vi "PIDAutoTune_ClosedLoopStep.vi"(7 "Configuration Parameters":T2={"Controller Constant Type"=enum."Ziegler Nicols - Normal", "Type of Controller"=enum."PI", "CO Offset"=0.25, "Kn"=1.0, "Tuning Tolerance"=0.001, "Plant Tolerance"=0.001, "Newest Avg Time "=1, "Long Ave Time"=6}, 8 "Sampling Time dt (s)":dbl=0.02, 9 "Tune":bool, 10 "Measurement  (PV)":dbl, 11 "Control Output (Co)":dbl) -> (0 "Plant and Test Data":T4, 1 "New Tuning Parameters":T3, 2 "Tuning Done":bool, 3 "Adj CO":dbl, 4 "Error Occured":bool, 6 "Diagnostic":T1)   [LabVIEW 2019, in "Trajectory_Library.lvlib"]
doc: "This routine can be used to make a step change to a PID control loop, track the results, and calculate PID tuning parameters. It wraps the NI LabVIEW PID auto-tuning functions for use with the WPILIB LabVIEW Math PID. This uses the CLOSED LOOP STEP type of test. \n\nWarning -- This routine will modify the control output. Use it in such a manner to be able to stop the tuning if problems occur -- like running out of field space while tuning a drive motor. \n\nInputs:\n -- Configuration Parameters -- cluster -- This contains the parameters defining the conditions of the test. Use the Pack routine to create this data cluster.\n -- Control Output -- double -- The Control Output (CO) value from the output of the PID to be tuned.\n -- Measurement (PV) -- double -- The Process Variable (PV) value used by the PID to be tuned.\n -- Tune -- boolean -- When TRUE, tuning is performed..\n -- Sampling time -- double -- Loop time in seconds. How fast the PID and this autotune function are executed. (Optional: Default 0.02 seconds) \n\nOutputs:\n -- Adj CO -- double -- The adjusted CO. This is sent to the actuator. (This vi is put between the PID and the actuator device)\n -- Tuning Done -- boolean -- This is set to TRUE when tuning has completed. Depending on the PV noise, tuning may never be \"DONE\". However if the new tuning parameters are relatively constant, they can still be used.\n -- New Tuning Parameters -- cluster --- Data cluster containing the calculated PID tuning parameters. \n -- Plant and Test Data -- cluster -- Data cluster containing information describing the transfer function of the system being controlled (Plant).\n -- Error Occured -- Boolean -- If TRUE, an error occured.\n -- Diagnostic Info -- cluster -- This contains additional information about the test being perfromed."
uses:
  Trajectory_Library.lvlib
  Timer_New.vi
  LinearFilter_ResetToValue.vi
  LinearFilter_Calculate.vi
  <vilib>/Utility/semaphor.llb/Obtain Semaphore Reference.vi
  Timer_Reset.vi
  Timer_Start.vi
  Timer_Stop.vi
  Timer_HasPeriodPassedOnce.vi
  <vilib>/addons/control/pid/autopid.llb/PID Autotuning Design (Auto).vi
  <vilib>/addons/control/pid/autopid.llb/PID Autotuning Design (Chien-Hrones-Reswick).vi
  LinearFilter_MovingAverage.vi
  LinearFilter_LowPassBW1.vi
  LinearFilter_LowPassBW2.vi
  LinearFilter_HighPassBW1.vi
  LinearFilter_HighPassBW2.vi
  <vilib>/Analysis/Matrix/Numeric/Conversions/Array To Matrix - RA.vi
  <vilib>/addons/control/pid/NI_PID_autopid.lvlib
  <vilib>/ptbypt/NI_PtbyPt.lvlib
  <vilib>/Analysis/Matrix/NI_Matrix.lvlib
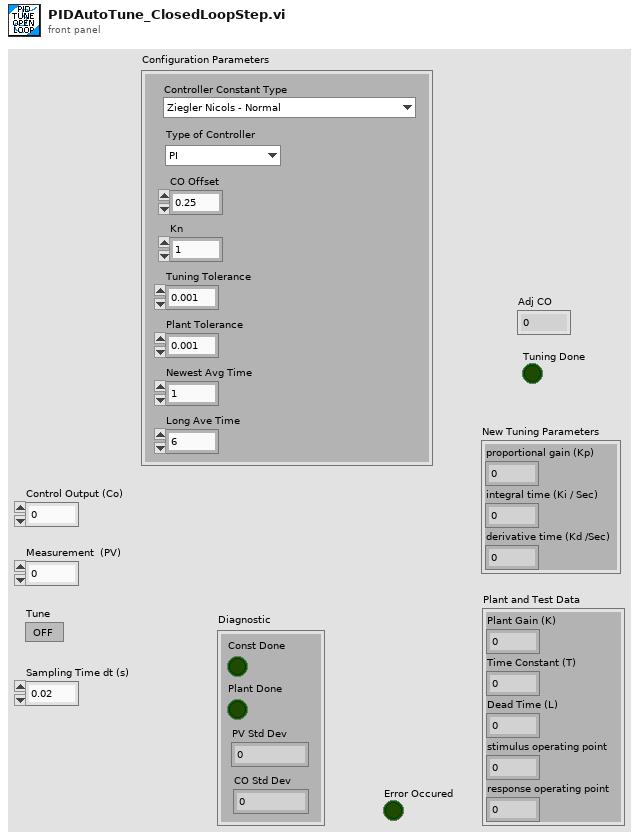
[diagram p1: front panel]
types:
  T1 = cluster{"Const Done":bool, "Plant Done":bool, "PV Std Dev":dbl, "CO Std Dev":dbl}
  T2 = cluster{"Controller Constant Type":enum16{"Ziegler Nicols - Fast", "Ziegler Nicols - Normal", "Ziegler Nicols - Slow", "CHR regulator - 0% overshoot", "CHR regulator - 20% overshoot", "CHR servo - 0 % overshoot", "CHR servo - 20% overshoot"}, "Type of Controller":enum16{"P", "PI", "PID"}, "CO Offset":dbl, "Kn":dbl, "Tuning Tolerance":dbl, "Plant Tolerance":dbl, "Newest Avg Time ":i32, "Long Ave Time":i32}
  T3 = cluster{"proportional gain (Kp)":dbl, "integral time (Ki / Sec)":dbl, "derivative time (Kd /Sec)":dbl}
  T4 = cluster{"Plant Gain (K)":dbl, "Time Constant (T)":dbl, "Dead Time (L)":dbl, "stimulus operating point":dbl, "response operating point":dbl}
  T5 = enum16{"Ziegler Nicols - Fast", "Ziegler Nicols - Normal", "Ziegler Nicols - Slow", "CHR regulator - 0% overshoot", "CHR regulator - 20% overshoot", "CHR servo - 0 % overshoot", "CHR servo - 20% overshoot"}
  T6 = cluster{"proportional gain (Kc)":dbl, "integral time (Ti, min)":dbl, "derivative time (Td, min)":dbl}
  T7 = cluster{"Plant Gain (K)":dbl, "Time Constant (T)":dbl, "Dead Time (L)":dbl}
  T8 = cluster{"Plant Gain (K)":dbl, "Time Constant (T)":dbl, "Dead Time (L)":dbl, "stimulus offset":dbl, "response offset":dbl}
  T9 = typedef "NI_Matrix.lvlib/RealMatrix.ctl" = dbl[][]
  T10 = cluster{"WithinTolerance":bool, "WithinTolerance":bool, "standard deviation":dbl, "standard deviation":dbl}
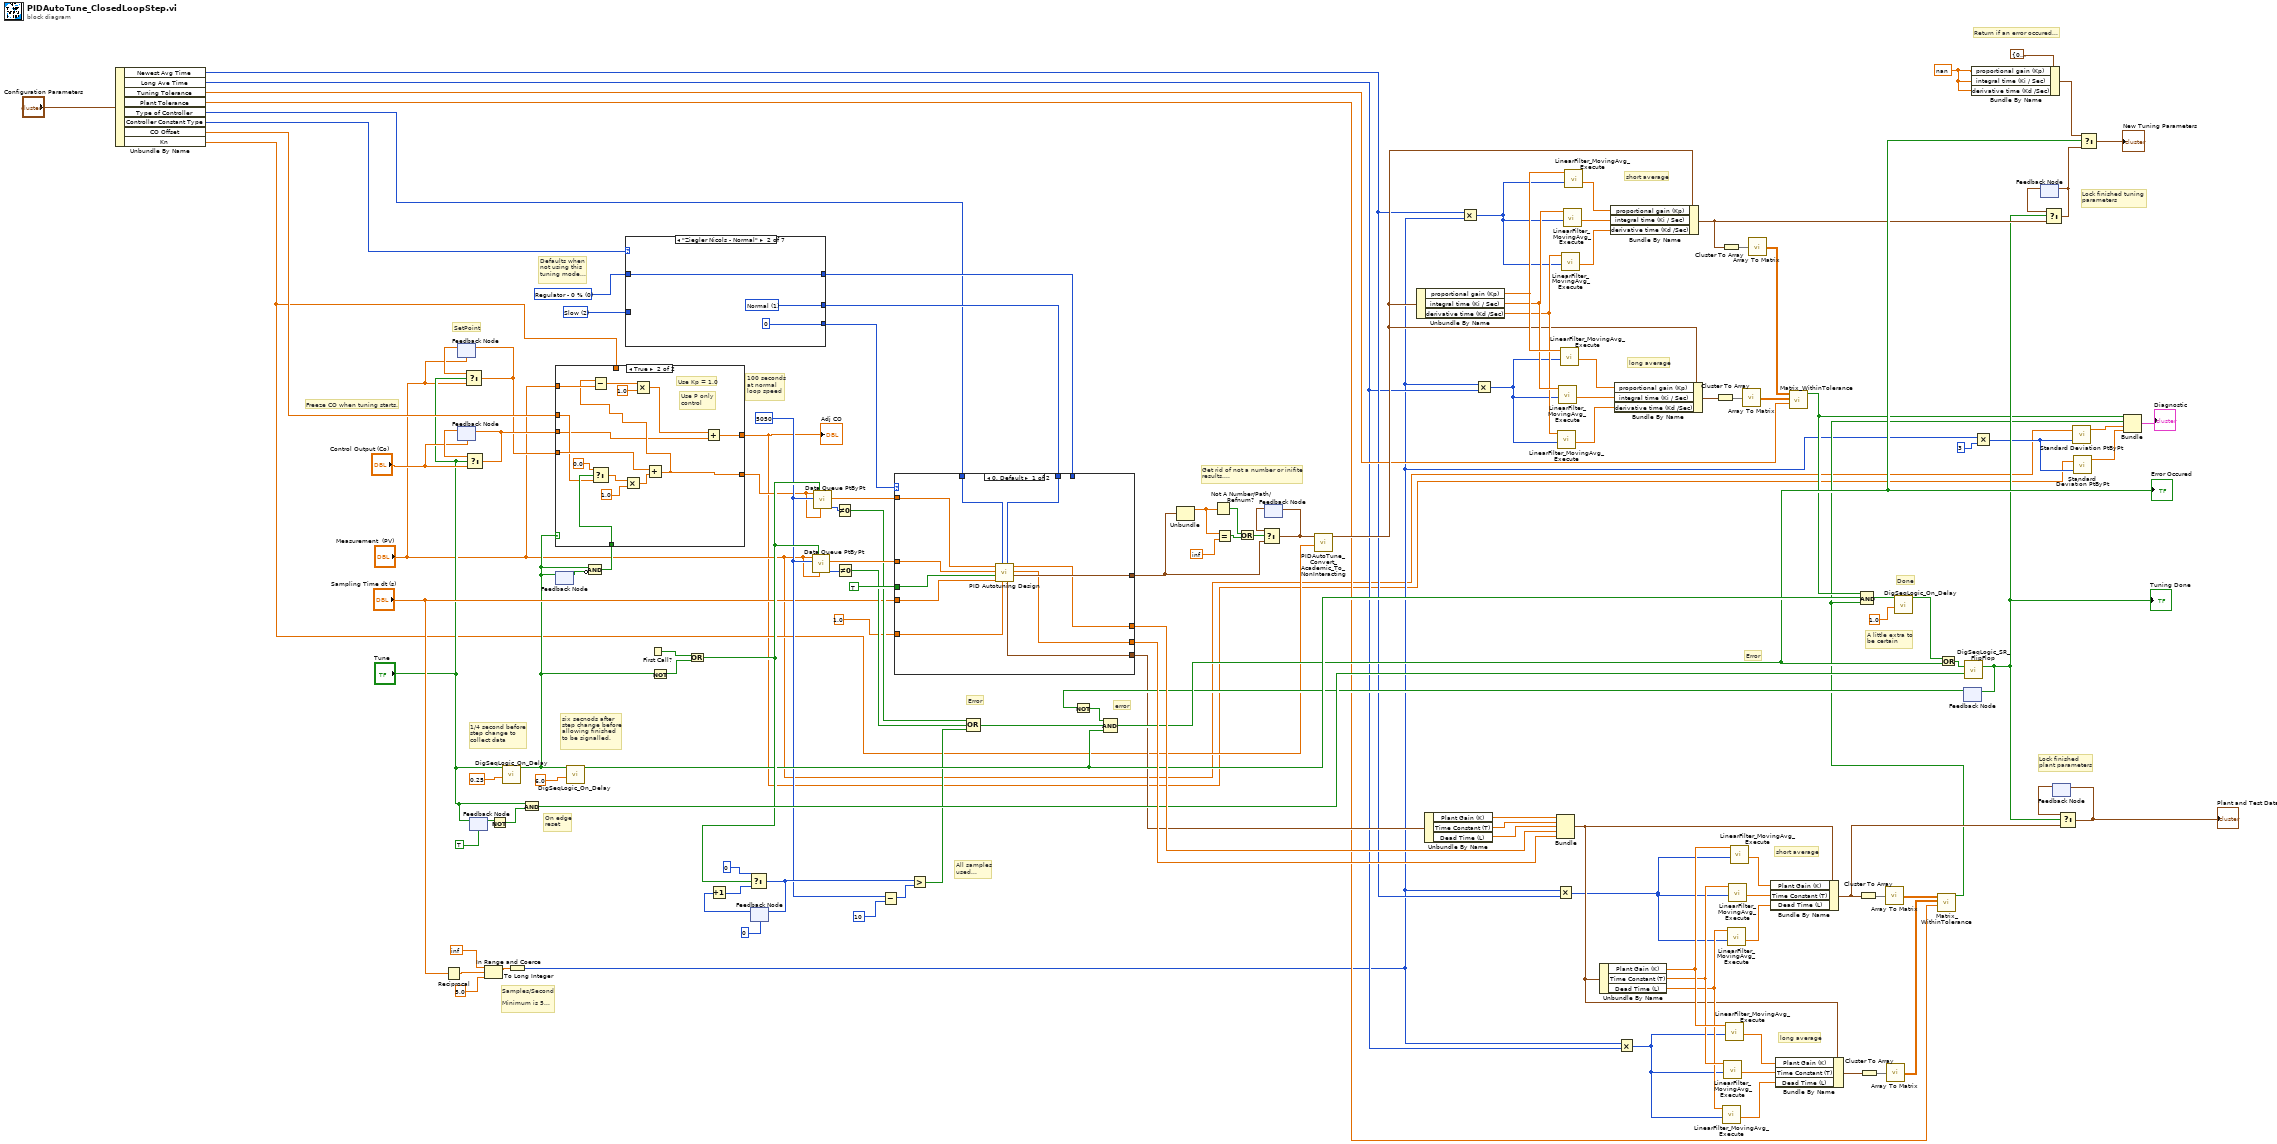
[diagram p0: block diagram]
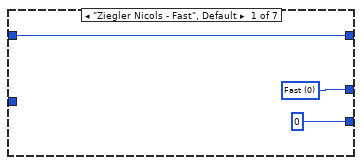
[diagram p2: hidden frame]
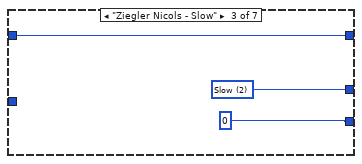
[diagram p3: hidden frame]
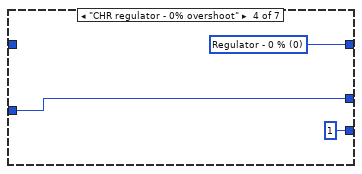
[diagram p4: hidden frame]
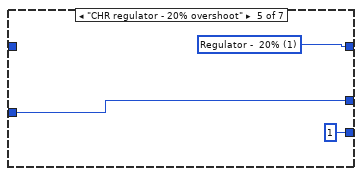
[diagram p5: hidden frame]
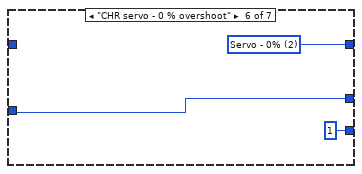
[diagram p6: hidden frame]
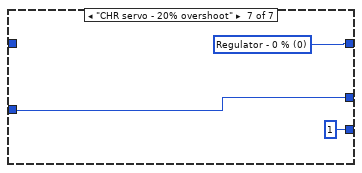
[diagram p7: hidden frame]
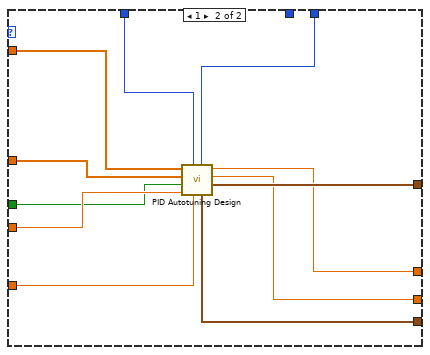
[diagram p8: hidden frame]
diagram:
  w89 = nan
  w104 = u16 2 items=["Fast", "Normal", "Slow"] ("Ziegler-Nichols Speed")
  w105 = u16 0 items=["Regulator - 0 %", "Regulator -  20%", "Servo - 0%", "Servo - 20%"] ("Tuning specifications")
  w76 = 5050 ("sample length")
  # "SetPoint"
  # "Get rid of not a number or inifite\nresults...."
  # "On edge\nreset"
  # "Error"
  # "All samples\nused..."
  # "Error"
  # "Done"
  # "Lock finished \nplant parameters"
  # "Lock finished tuning\nparameters"
  # "Samples/Second\n\nMinimum is 5..."
  # "long average"
  # "short average"
  # "long average"
  # "short average"
  # "error"
  # "Return if an error occured..."
  # "A little extra to\nbe certain"
  # "Defaults when\nnot using this\ntuning mode..."
  # "100 seconds\nat normal\nloop speed"
  # "Freeze CO when tuning starts."
  # "six secnods after\nstep change before\nallowing finished \nto be signalled."
  # "1/4 second before\nstep change to\ncollect data"
  n1 = Unbundle By Name("Configuration Parameters") -> ("Newest Avg Time"=w21:i32, "Long Ave Time"=w20:i32, "Tuning Tolerance"=w26:dbl, "Plant Tolerance"=w25:dbl, "Type of Controller"=w28:enum16{"P", "PI", "PID"}, "Controller Constant Type"=w29:T5, "CO Offset"=w27:dbl, "Kn"=w9:dbl)
  n2 = Reciprocal(x="Sampling Time dt (s)") -> (1/x=w66:dbl)
  n3 = feedback #1("Measurement  (PV)") -> (w16:dbl)
  n4 = feedback #2("Control Output (Co)") -> (w119:dbl)
  n5 = Select(t=w16, s="Tune", f="Measurement  (PV)") -> (s? t:f=w14:dbl)
  n6 = feedback-in #1(w14) -> ()
  n7 = Select(t=w119, s="Tune", f="Control Output (Co)") -> (s? t:f=w120:dbl)
  n8 = feedback-in #2(w120) -> ()
  n9 = feedback-in #3("Tune") -> ()
  n10 = feedback #3(TRUE ("Tune")) -> (w116:bool)
  n11 = In Range and Coerce(upper limit=inf, x=w66, lower limit=5.0) -> (coerced(x)=w57:dbl)  [unwired: 1 out]
  n12 = Not(x=w116) -> (.not. x?=w115:bool)
  n13 = call "DigSeqLogic_On_Delay.vi"("Delay"=0.25, "Input"="Tune") -> ("Output"=w10:bool)  [unwired: 8 in, 1 out]
  n14 = To Long Integer(number=w57) -> (32bit integer=w5:i32)
  n15 = And(x="Tune", y=w115) -> (x .and. y?=w114:bool)
  n16 = feedback-in #4(w10) -> ()
  n17 = feedback #4() -> (w13:bool)  [unwired: 1 in]
  n18 = call "DigSeqLogic_On_Delay.vi"("Delay"=6.0, "Input"=w10) -> ("Output"=w83:bool)  [unwired: 8 in, 1 out]
  n19 = Compound Arithmetic op=AND(w10, invert w13) -> (w12:bool)
  n20 = case shown="True" w10 {
    tunnel: w120 -> [w135 w140]
    tunnel: w27 -> [_ w141]
    tunnel: [w135 w146] -> w1
    tunnel: w14 -> [w134 w143]
    tunnel: "Measurement  (PV)" -> [_ w149]
    tunnel: w12 -> [_ w144]
    tunnel: [w134 w142] -> w11
    tunnel: w9 -> [_ _]
    frame False {
    }
    frame True {
      # "Use P only \ncontrol"
      # "Use Kp = 1.0"
      n21 = Select(t=0.0, s=w144, f=w141) -> (s? t:f=w137:dbl)
      n22 = Multiply(x=w137, y=1.0) -> (x*y=w139:dbl)
      n23 = Add(x=w143, y=w139) -> (x+y=w142:dbl)
      n24 = Subtract(x=w142, y=w149) -> (x-y=w148:dbl)
      n25 = Multiply(x=w148, y=1.0) -> (x*y=w147:dbl)
      n26 = Add(x=w147, y=w140) -> (x+y=w146:dbl)
    }
  }
  "Adj CO" <- w1
  n27 = case shown="\"Ziegler Nicols - Normal\"" w29 {
    tunnel: [w152 w155 w158 w159 w162 w165 w168] -> w108
    tunnel: [0 0 0 1 1 1 1] -> w107
    tunnel: [w150 w153 w156 w160 w163 w166 w169] -> w106
    tunnel: w105 -> [w150 w153 w156 _ _ _ _]
    tunnel: w104 -> [_ _ _ w159 w162 w165 w168]
    frame "Ziegler Nicols - Fast", Default {
      w152 = u16 0 items=["Fast", "Normal", "Slow"] ("Ziegler-Nichols Speed")
    }
    frame "Ziegler Nicols - Normal" {
      w155 = u16 1 items=["Fast", "Normal", "Slow"] ("Ziegler-Nichols Speed")
    }
    frame "Ziegler Nicols - Slow" {
      w158 = u16 2 items=["Fast", "Normal", "Slow"] ("Ziegler-Nichols Speed")
    }
    frame "CHR regulator - 0% overshoot" {
      w160 = u16 0 items=["Regulator - 0 %", "Regulator -  20%", "Servo - 0%", "Servo - 20%"] ("Tuning specifications")
    }
    frame "CHR regulator - 20% overshoot" {
      w163 = u16 1 items=["Regulator - 0 %", "Regulator -  20%", "Servo - 0%", "Servo - 20%"] ("Tuning specifications")
    }
    frame "CHR servo - 0 % overshoot" {
      w166 = u16 2 items=["Regulator - 0 %", "Regulator -  20%", "Servo - 0%", "Servo - 20%"] ("Tuning specifications")
    }
    frame "CHR servo - 20% overshoot" {
      w169 = u16 0 items=["Regulator - 0 %", "Regulator -  20%", "Servo - 0%", "Servo - 20%"] ("Tuning specifications")
    }
  }
  n28 = First Call?() -> (First Call?: T/F=w88:bool)
  n29 = Not(x=w10) -> (.not. x?=w87:bool)
  n30 = Or(x=w88, y=w87) -> (x .or. y?=w85:bool)
  n31 = feedback #5(0) -> (w80:i32)
  n32 = Increment(x=w80) -> (x+1=w79:i32)
  n33 = Select(t=0, s=w85, f=w79) -> (s? t:f=w78:i32)
  n34 = feedback-in #5(w78) -> ()
  n35 = call <vilib>:"Data Queue PtByPt.vi"("initial queue element"="Measurement  (PV)", "initialize"=w85, "sample length"=w76, "input data point"="Measurement  (PV)") -> ("error"=w96:i32, "Current Queue"=w128:dbl[])  [unwired: 3 in, 3 out]
  n36 = call <vilib>:"Data Queue PtByPt.vi"("initial queue element"=w11, "initialize"=w85, "sample length"=w76, "input data point"=w11) -> ("error"=w97:i32, "Current Queue"=w129:dbl[])  [unwired: 3 in, 3 out]
  n37 = Not Equal To 0?(x=w97) -> (x != 0?=w73:bool)
  n38 = Not Equal To 0?(x=w96) -> (x != 0?=w72:bool)
  n39 = Subtract(x=w76, y=10) -> (x-y=w77:i32)
  n40 = case shown="0, Default" w107 {
    tunnel: [w181 w192] -> w132
    tunnel: "Sampling Time dt (s)" -> [w180 w191]
    tunnel: w129 -> [w179 w190]
    tunnel: w128 -> [w178 w189]
    tunnel: w28 -> [w177 w188]
    tunnel: [w171 w187] -> w38
    tunnel: [w176 w186] -> w124
    tunnel: [w175 w185] -> w123
    tunnel: 1.0 ("Kn") -> [w174 w184]
    tunnel: w108 -> [w173 _]
    tunnel: w106 -> [_ w183]
    tunnel: TRUE ("closed-loop?") -> [w172 w182]
    frame 0, Default {
      n41 = call-poly <vilib>:"PID Autotuning Design.vi"("Ziegler-Nichols Speed"=w173, "Controller Gain (K)"=w174, "Type of Controller"=w177, "dt (s)"=w180, "closed-loop?"=w172, "Response signal"=w178, "Stimulus signal"=w179) -> ("PID gains"=w181:T6, "response operating point"=w175:dbl, "stimulus operating point"=w176:dbl, "Plant Parameters"=w171:T7)  [unwired: 1 in]
    }
    frame 1 {
      n42 = call-poly <vilib>:"PID Autotuning Design.vi"("Tuning specifications"=w183, "Controller Gain (K)"=w184, "Type of Controller"=w188, "dt (s)"=w191, "closed-loop?"=w182, "Response signal"=w189, "Stimulus signal"=w190) -> ("PID gains"=w192:T6, "response offset"=w185:dbl, "stimulus offset"=w186:dbl, "Plant Parameters"=w187:T7)  [unwired: 1 in]
    }
  }
  n43 = Greater?(x=w78, y=w77) -> (0:w74:bool)
  n44 = Compound Arithmetic op=OR(w73, w72, w74) -> (w84:bool)
  n45 = Unbundle(w132) -> ("proportional gain (Kc)"=w69:dbl)  [unwired: 2 out]
  n46 = Not A Number/Path/Refnum?(number/path/refnum=w69) -> (NaN/Path/Refnum?=w68:bool)
  n47 = Equal?(x=w69, y=inf) -> (x = y?=w98:bool)
  n48 = Or(x=w68, y=w98) -> (x .or. y?=w99:bool)
  n49 = feedback #6() -> (w131:T6)  [unwired: 1 in]
  n50 = Select(t=w131, s=w99, f=w132) -> (s? t:f=w133:T6)
  n51 = feedback-in #6(w133) -> ()
  n52 = call "PIDAutoTune_Convert_Academic_To_NonInteracting.vi"("Kn"=w9, "PID gains NI Academic"=w133) -> ("PID Gains Non Interacting"=w53:T3)  [unwired: 9 in]
  n53 = Unbundle By Name(w53) -> ("proportional gain (Kp)"=w60:dbl, "integral time (Ki / Sec)"=w59:dbl, "derivative time (Kd /Sec)"=w58:dbl)
  n54 = Unbundle By Name(w38) -> ("Plant Gain (K)"=w127:dbl, "Time Constant (T)"=w126:dbl, "Dead Time (L)"=w125:dbl)
  n55 = Multiply(x=w21, y=w5) -> (x*y=w24:i32)
  n56 = Multiply(x=w5, y=w20) -> (x*y=w56:i32)
  n57 = Bundle("Plant Gain (K)"=w127, "Time Constant (T)"=w126, "Dead Time (L)"=w125, "stimulus offset"=w124, "response offset"=w123) -> (w37:T8)  [unwired: 1 in]
  n58 = Multiply(x=w5, y=w21) -> (x*y=w22:i32)
  n59 = call "LinearFilter_MovingAvg_Execute.vi"("Samples"=w56, "Input"=w58) -> ("Output"=w61:dbl)  [unwired: 9 in]
  n60 = call "LinearFilter_MovingAvg_Execute.vi"("Samples"=w56, "Input"=w59) -> ("Output"=w63:dbl)  [unwired: 9 in]
  n61 = call "LinearFilter_MovingAvg_Execute.vi"("Samples"=w56, "Input"=w60) -> ("Output"=w62:dbl)  [unwired: 9 in]
  n62 = call "LinearFilter_MovingAvg_Execute.vi"("Samples"=w24, "Input"=w58) -> ("Output"=w100:dbl)  [unwired: 9 in]
  n63 = call "LinearFilter_MovingAvg_Execute.vi"("Samples"=w24, "Input"=w59) -> ("Output"=w101:dbl)  [unwired: 9 in]
  n64 = call "LinearFilter_MovingAvg_Execute.vi"("Samples"=w24, "Input"=w60) -> ("Output"=w102:dbl)  [unwired: 9 in]
  n65 = Unbundle By Name(w37) -> ("Plant Gain (K)"=w42:dbl, "Time Constant (T)"=w41:dbl, "Dead Time (L)"=w40:dbl)
  n66 = Bundle By Name(cluster=w53, "proportional gain (Kp)"=w102, "integral time (Ki / Sec)"=w101, "derivative time (Kd /Sec)"=w100) -> (w52:T3)
  n67 = Bundle By Name(cluster=w53, "proportional gain (Kp)"=w62, "integral time (Ki / Sec)"=w63, "derivative time (Kd /Sec)"=w61) -> (w55:T3)
  n68 = Multiply(x=w5, y=w20) -> (x*y=w39:i32)
  n69 = Cluster To Array(cluster=w55) -> (array=w54:dbl[])
  n70 = Cluster To Array(cluster=w52) -> (array=w51:dbl[])
  n71 = call "LinearFilter_MovingAvg_Execute.vi"("Samples"=w39, "Input"=w40) -> ("Output"=w43:dbl)  [unwired: 9 in]
  n72 = call "LinearFilter_MovingAvg_Execute.vi"("Samples"=w39, "Input"=w41) -> ("Output"=w45:dbl)  [unwired: 9 in]
  n73 = call "LinearFilter_MovingAvg_Execute.vi"("Samples"=w39, "Input"=w42) -> ("Output"=w44:dbl)  [unwired: 9 in]
  n74 = call "LinearFilter_MovingAvg_Execute.vi"("Samples"=w22, "Input"=w40) -> ("Output"=w46:dbl)  [unwired: 9 in]
  n75 = call "LinearFilter_MovingAvg_Execute.vi"("Samples"=w22, "Input"=w41) -> ("Output"=w47:dbl)  [unwired: 9 in]
  n76 = call "LinearFilter_MovingAvg_Execute.vi"("Samples"=w22, "Input"=w42) -> ("Output"=w48:dbl)  [unwired: 9 in]
  n77 = call-poly <vilib>:"Array To Matrix.vi"("Real 1D Array"=w54) -> ("Real Matrix (Column Vector)"=w50:T9)
  n78 = call-poly <vilib>:"Array To Matrix.vi"("Real 1D Array"=w51) -> ("Real Matrix (Column Vector)"=w49:T9)
  n79 = Bundle By Name(cluster=w37, "Plant Gain (K)"=w48, "Time Constant (T)"=w47, "Dead Time (L)"=w46) -> (w33:T8)
  n80 = Bundle By Name(cluster=w37, "Plant Gain (K)"=w44, "Time Constant (T)"=w45, "Dead Time (L)"=w43) -> (w34:T8)
  n81 = call "Matrix_WithinTolerance.vi"("Tolerance"=w26, "Matrix B"=w50, "Matrix A"=w49) -> ("WithinTolerance"=w18:bool)  [unwired: 7 in, 1 out]
  n82 = Cluster To Array(cluster=w33) -> (array=w36:dbl[])
  n83 = Cluster To Array(cluster=w34) -> (array=w35:dbl[])
  n84 = call-poly <vilib>:"Array To Matrix.vi"("Real 1D Array"=w36) -> ("Real Matrix (Column Vector)"=w32:T9)
  n85 = call-poly <vilib>:"Array To Matrix.vi"("Real 1D Array"=w35) -> ("Real Matrix (Column Vector)"=w31:T9)
  n86 = call "Matrix_WithinTolerance.vi"("Tolerance"=w25, "Matrix B"=w31, "Matrix A"=w32) -> ("WithinTolerance"=w17:bool)  [unwired: 7 in, 1 out]
  n87 = Compound Arithmetic op=AND(w18, w83, w17) -> (w110:bool)
  n88 = call "DigSeqLogic_On_Delay.vi"("Delay"=1.0, "Input"=w110) -> ("Output"=w94:bool)  [unwired: 8 in, 1 out]
  n89 = feedback #7() -> (w70:bool)  [unwired: 1 in]
  n90 = Not(x=w70) -> (.not. x?=w71:bool)
  n91 = Compound Arithmetic op=AND(w71, w84, w83) -> (w82:bool)
  "Error Occured" <- w82
  n92 = Or(x=w94, y=w82) -> (x .or. y?=w95:bool)
  n93 = call "DigSeqLogic_SR_FlipFlop.vi"("Set"=w95, "Reset"=w114) -> ("Output"=w23:bool)  [unwired: 12 in, 1 out]
  "Tuning Done" <- w23
  n94 = feedback-in #7(w23) -> ()
  n95 = Bundle By Name(cluster=T3 {"proportional gain (Kp)"=0.0, "integral time (Ki / Sec)"=0.0, "derivative time (Kd /Sec)"=0.0} ("t"), "proportional gain (Kp)"=w89, "integral time (Ki / Sec)"=w89, "derivative time (Kd /Sec)"=w89) -> (w90:T3)
  n96 = Multiply(x=w5, y=3) -> (x*y=w6:i32)
  n97 = feedback #8() -> (w111:T3)  [unwired: 1 in]
  n98 = Select(t=w111, s=w23, f=w52) -> (s? t:f=w92:T3)
  n99 = feedback-in #8(w92) -> ()
  n100 = feedback #9() -> (w112:T8)  [unwired: 1 in]
  n101 = Select(t=w112, s=w23, f=w33) -> (s? t:f=w113:T8)
  "Plant and Test Data" <- w113
  n102 = feedback-in #9(w113) -> ()
  n103 = call <vilib>:"Standard Deviation PtByPt.vi"("x"="Measurement  (PV)", "sample length"=w6) -> ("standard deviation"=w4:dbl)  [unwired: 1 in, 2 out]
  n104 = call <vilib>:"Standard Deviation PtByPt.vi"("x"=w1, "sample length"=w6) -> ("standard deviation"=w3:dbl)  [unwired: 1 in, 2 out]
  n105 = Select(t=w90, s=w82, f=w92) -> (s? t:f=→"New Tuning Parameters":T3)
  n106 = Bundle("WithinTolerance"=w18, "WithinTolerance"=w17, "standard deviation"=w4, "standard deviation"=w3) -> (→"Diagnostic":T10)  [unwired: 1 in]
